vi "Get VI Name.vi"(11 "Parametric VI Call In":refnum<class "Parametric VI Call.lvclass">) -> (2 "VI Name":string)   [LabVIEW 2020, in "Parametric VI Call.lvclass"]
uses:
  Parametric VI Call.lvclass
  Parametric VI Call.lvclass/Parametric VI Call.ctl
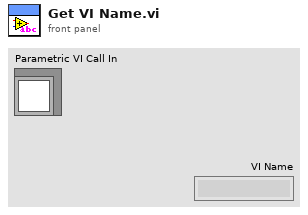
[diagram p1: front panel]
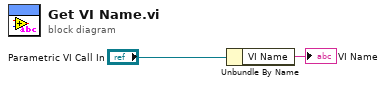
[diagram p0: block diagram]
diagram:
  n1 = Unbundle By Name("Parametric VI Call In") -> ("VI Name"=→"VI Name":string)
